vi "Paths.vi"(7 "error constant":errorcluster, 10 "file path (dialog if empty)":path) -> (0 "error IO":errorcluster, 1 "limits file path":path, 2 "File Names":string[](array[string]), 3 "All MCS Registers":cluster{"all rows":string[][]}[](array[cluster]), 4 "Calibration date file path":path, 5 "Email settings file path":path, 6 "Users Db":path, 8 "Limit of rate change path":path, 9 "Offsets file path":path)   [LabVIEW 2025]
uses:
  CTRLS/GLB_VAR.vi
  mcs/Tachometer_MAIN Folder/CTRLS/New/MCS Tag.ctl
  CTRLS/New/Monitiring MCS Tags.ctl
  CTRLS/New/Mcs All Tags Registers.ctl
  <vilib>/Utility/file.llb/Read Delimited Spreadsheet (string).vi
panel:
  out "Array 5":string[][](array[string])
  out "Array 4":string[][](array[string])
  out "Array 3":string[][](array[string])
  out "Array 2":i32[](array[numeric])
  out "Array":i32[](array[numeric])
  out "Register":string[](array[string])
  out "Name":string[](array[string])
  out "Application Directory":path
  out "Templates directory":path
  out "config file path":path
  out "Test Setups directory":path
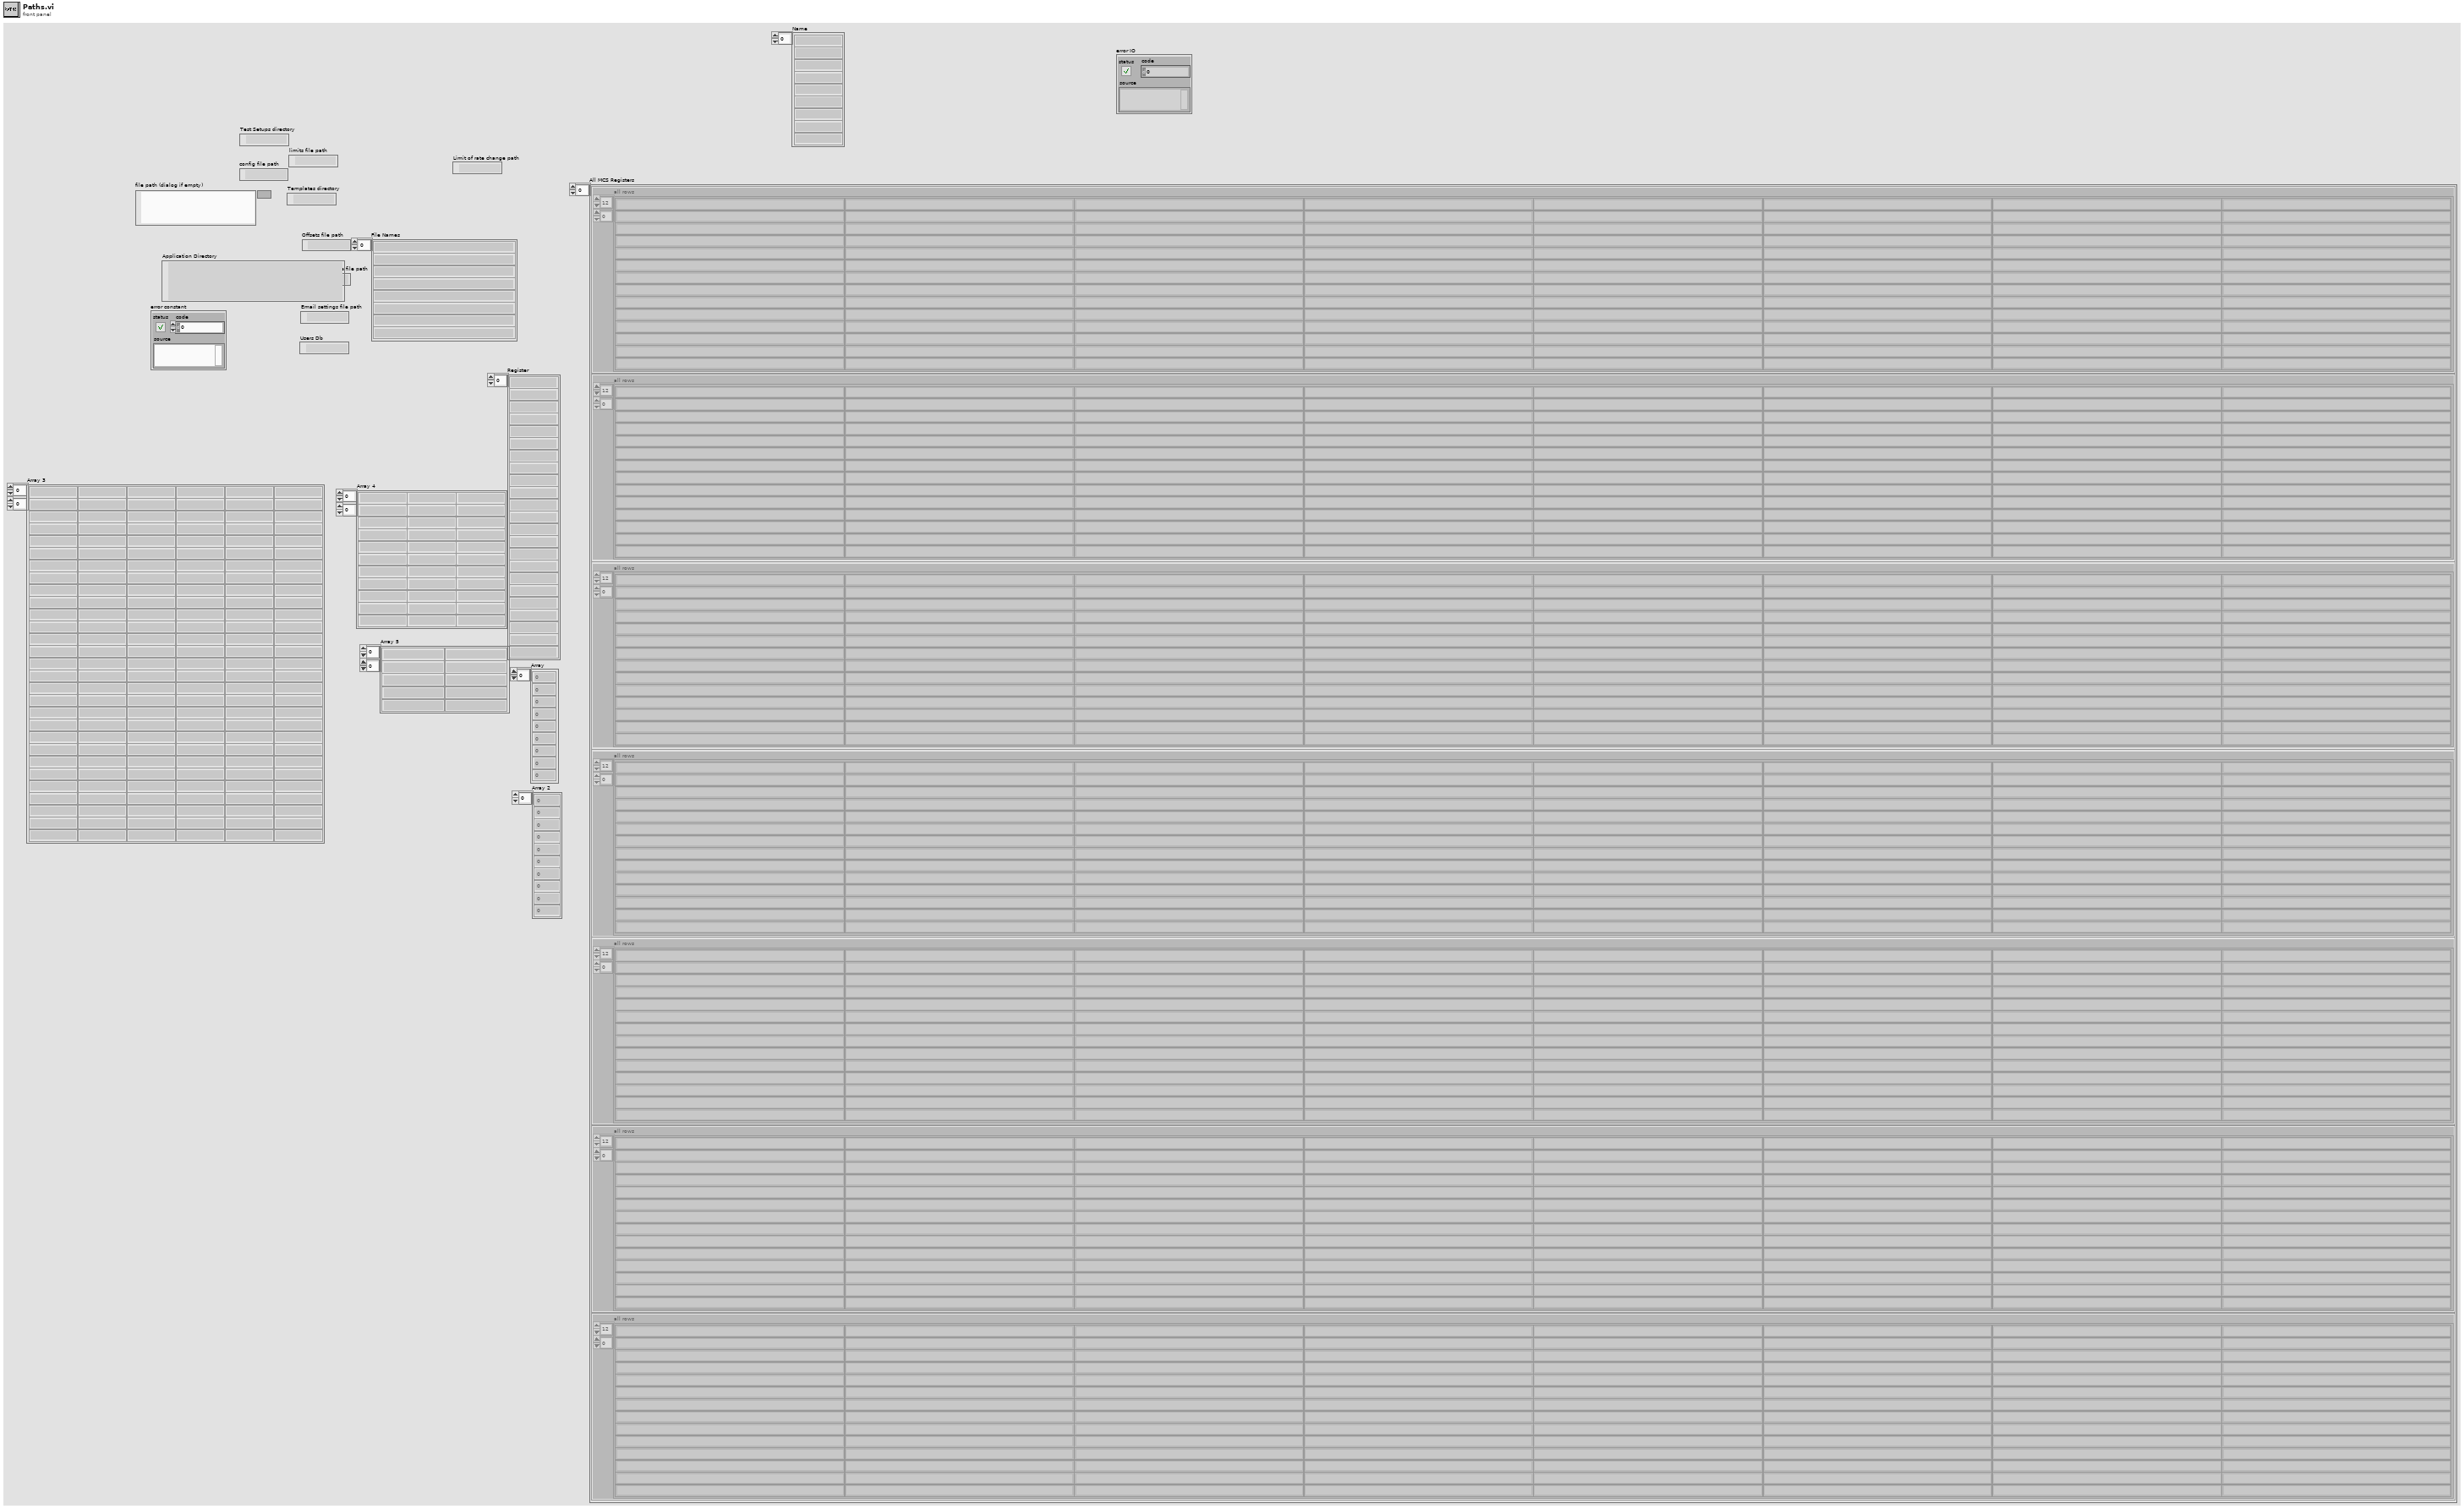
[diagram p1: front panel]
types:
  T1 = typedef "Mcs All Tags Registers.ctl" = cluster{"Suction addr":i32[][], "Discharge addr":i32[][], "Loging addr":i32[][], "Monitiring MCS Tags":T2, "Monitiring MCS Coils":cluster{"Tag Name":string, "Modbus Input Register":sgl, "Value":bool}[][]}
  T2 = typedef "Monitiring MCS Tags.ctl" = T3[][]
  T3 = typedef "MCS Tag.ctl" = cluster{"Tag Name":string, "Modbus Input Register":sgl, "Value":sgl}
  T4 = cluster{"Tag Name":string, "Modbus Input Register":sgl, "Value":bool}[][]
  T5 = enum16{"open", "replace", "create", "open or create", "replace or create", "replace or create with confirmation"}
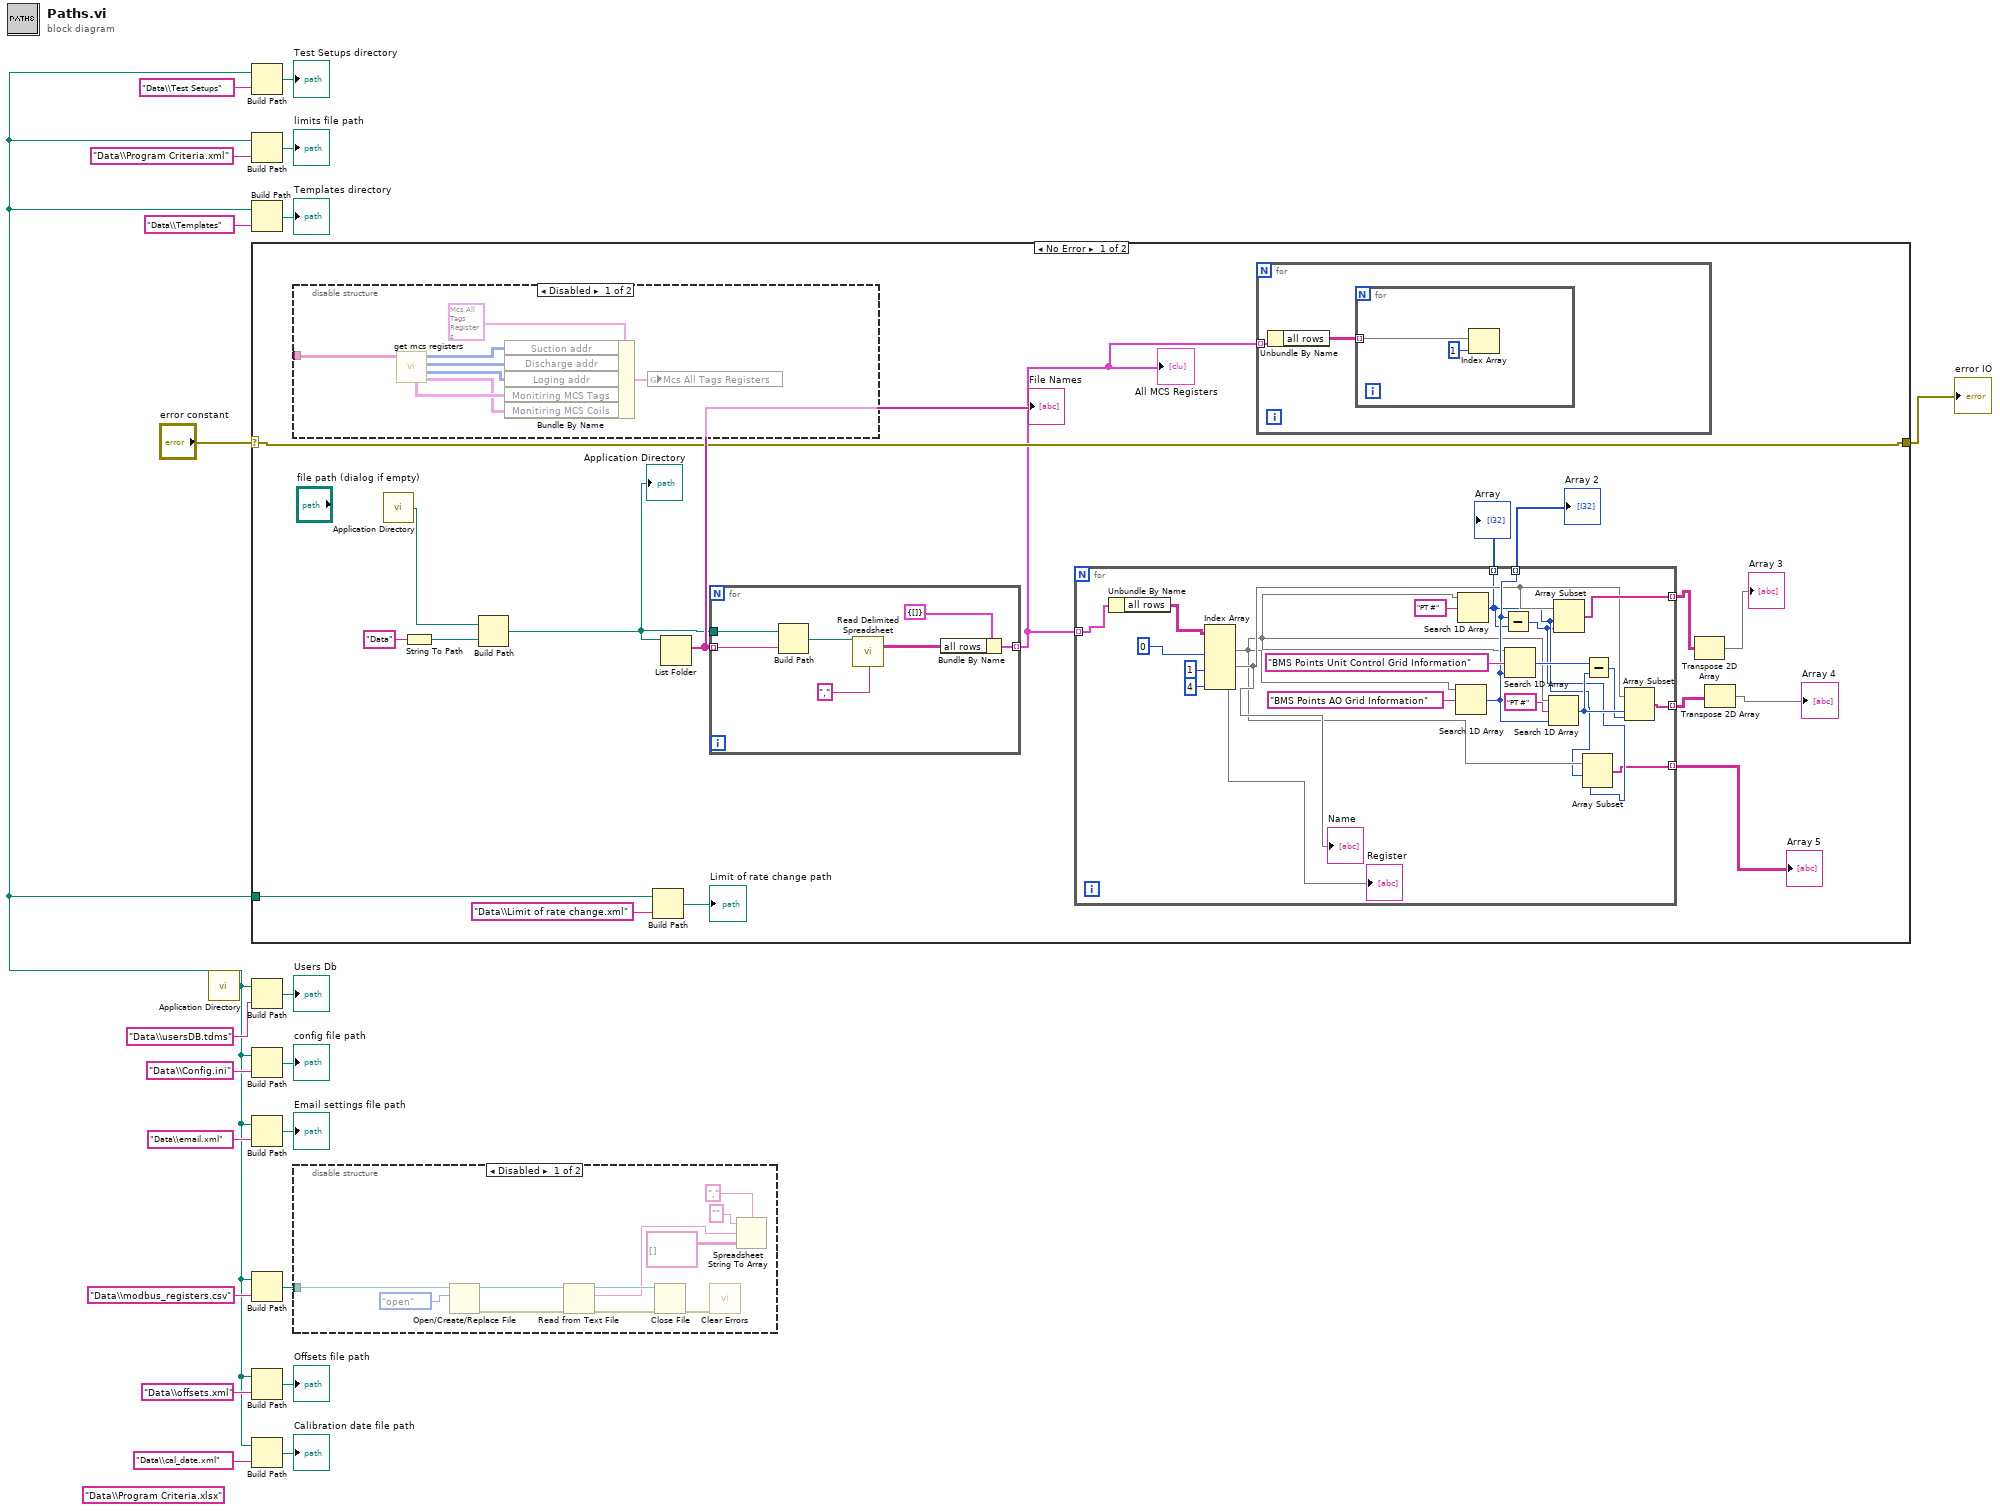
[diagram p0: block diagram]
diagram:
  (unwired) "Data\\Program Criteria.xlsx"
  n1 = call <vilib>:"Application Directory.vi"() -> ("Application Directory"=w4:path)
  n2 = Build Path(base path=w4, name or relative path="Data\\Test Setups") -> (appended path=→"Test Setups directory":path)
  n3 = Build Path(base path=w4, name or relative path="Data\\Program Criteria.xml") -> (appended path=→"limits file path":path)
  n4 = Build Path(base path=w4, name or relative path="Data\\Templates") -> (appended path=→"Templates directory":path)
  n5 = case shown="No Error" "error constant" {
    selector: "error constant" -> [w31 w79]
    tunnel: w4 -> [w36 _]
    tunnel: [w31 w79] -> w1
    frame No Error {
      n6 = disable-structure shown="Disabled" {
        disable-tunnel: _ -> [w75 _]
        frame Disabled {
          n7 = call "get mcs registers.vi"("MCS CSV"=w75) -> ("coils"=w73:T4, "Array 2"=w76:i32[][], "Array 3"=w77:i32[][], "Array 4"=w78:i32[][], "Array"=w74:T3[][])  [unwired: 6 in]
          n8 = Bundle By Name(cluster=T1 {"Suction addr"=[[30003, 30004, 30005, 30006], [30011, 30012, 30016, 30017], [30098, 30103, 30108, 30113], [30101, 30106, 30111, 30116]], "Discharge addr"=[[30007, 30008, 30009, 30010], [30018, 30019, 30020, 30021], [30099, 30104, 30109, 30114], [30100, 30105, 30110, 30115]], "Loging addr"=[[30093, 30094, 30095, 30096, 0, 0], [30097, 30102, 30107, 30112, 0, 0], [30087, 30088, 30089, 30090, 30091, 30092], [30036, 30037, 30038, 30039, 0, 0], [30001, 30002, 0, 0, 0, 0], [30044, 30045, 0, 0, 0, 0], [30117, 30118, 30119, 0, 0, 0], [30022, 30023, 30024, 30025, 30026, 30027]], "Monitiring MCS Tags"=[[{"Tag Name"="MP+OL1", "Modbus Input Register"=30028.0, "Value"=0.0}, {"Tag Name"="MP+OL2", "Modbus Input Register"=30029.0, "Value"=0.0}], [{"Tag Name"="MP+OL2", "Modbus Input Register"=30029.0, "Value"=0.0}, {"Tag Name"="MP+OL3", "Modbus Input Register"=30030.0, "Value"=0.0}], [{"Tag Name"="MP+OL3", "Modbus Input Register"=30030.0, "Value"=0.0}, {"Tag Name"="MP+OL4", "Modbus Input Register"=30031.0, "Value"=0.0}], [{"Tag Name"="MP+OL4", "Modbus Input Register"=30031.0, "Value"=0.0}, {"Tag Name"="OIL.LEVEL1", "Modbus Input Register"=30032.0, "Value"=0.0}], [{"Tag Name"="OIL.LEVEL1", "Modbus Input Register"=30032.0, "Value"=0.0}, {"Tag Name"="OIL.LEVEL2", "Modbus Input Register"=30033.0, "Value"=0.0}], [{"Tag Name"="OIL.LEVEL2", "Modbus Input Register"=30033.0, "Value"=0.0}, {"Tag Name"="OIL.LEVEL3", "Modbus Input Register"=30034.0, "Value"=0.0}], [{"Tag Name"="OIL.LEVEL3", "Modbus Input Register"=30034.0, "Value"=0.0}, {"Tag Name"="OIL.LEVEL4", "Modbus Input Register"=30035.0, "Value"=0.0}], [{"Tag Name"="OIL.LEVEL4", "Modbus Input Register"=30035.0, "Value"=0.0}, {"Tag Name"="PUMPDOWN1", "Modbus Input Register"=30040.0, "Value"=0.0}], [{"Tag Name"="PUMPDOWN1", "Modbus Input Register"=30040.0, "Value"=0.0}, {"Tag Name"="PUMPDOWN2", "Modbus Input Register"=30041.0, "Value"=0.0}], [{"Tag Name"="PUMPDOWN2", "Modbus Input Register"=30041.0, "Value"=0.0}, {"Tag Name"="PUMPDOWN3", "Modbus Input Register"=30042.0, "Value"=0.0}], [{"Tag Name"="PUMPDOWN3", "Modbus Input Register"=30042.0, "Value"=0.0}, {"Tag Name"="PUMPDOWN4", "Modbus Input Register"=30043.0, "Value"=0.0}], [{"Tag Name"="PUMPDOWN4", "Modbus Input Register"=30043.0, "Value"=0.0}, {"Tag Name"="COMP1", "Modbus Input Register"=30046.0, "Value"=0.0}], [{"Tag Name"="COMP1", "Modbus Input Register"=30046.0, "Value"=0.0}, {"Tag Name"="COMP2", "Modbus Input Register"=30050.0, "Value"=0.0}], [{"Tag Name"="COMP2", "Modbus Input Register"=30050.0, "Value"=0.0}, {"Tag Name"="COMP3", "Modbus Input Register"=30054.0, "Value"=0.0}], [{"Tag Name"="COMP3", "Modbus Input Register"=30054.0, "Value"=0.0}, {"Tag Name"="COMP4", "Modbus Input Register"=30058.0, "Value"=0.0}], [{"Tag Name"="COMP4", "Modbus Input Register"=30058.0, "Value"=0.0}, {"Tag Name"="LOADSOL1", "Modbus Input Register"=30047.0, "Value"=0.0}], [{"Tag Name"="LOADSOL1", "Modbus Input Register"=30047.0, "Value"=0.0}, {"Tag Name"="LOADSOL2", "Modbus Input Register"=30051.0, "Value"=0.0}], [{"Tag Name"="LOADSOL2", "Modbus Input Register"=30051.0, "Value"=0.0}, {"Tag Name"="LOADSOL3", "Modbus Input Register"=30055.0, "Value"=0.0}], [{"Tag Name"="LOADSOL3", "Modbus Input Register"=30055.0, "Value"=0.0}, {"Tag Name"="LOADSOL4", "Modbus Input Register"=30059.0, "Value"=0.0}], [{"Tag Name"="LOADSOL4", "Modbus Input Register"=30059.0, "Value"=0.0}, {"Tag Name"="UNLDSOL1", "Modbus Input Register"=30048.0, "Value"=0.0}], [{"Tag Name"="UNLDSOL1", "Modbus Input Register"=30048.0, "Value"=0.0}, {"Tag Name"="UNLDSOL2", "Modbus Input Register"=30052.0, "Value"=0.0}], [{"Tag Name"="UNLDSOL2", "Modbus Input Register"=30052.0, "Value"=0.0}, {"Tag Name"="UNLDSOL3", "Modbus Input Register"=30056.0, "Value"=0.0}], [{"Tag Name"="UNLDSOL3", "Modbus Input Register"=30056.0, "Value"=0.0}, {"Tag Name"="UNLDSOL4", "Modbus Input Register"=30060.0, "Value"=0.0}], [{"Tag Name"="UNLDSOL4", "Modbus Input Register"=30060.0, "Value"=0.0}, {"Tag Name"="ESV1", "Modbus Input Register"=30049.0, "Value"=0.0}], [{"Tag Name"="ESV1", "Modbus Input Register"=30049.0, "Value"=0.0}, {"Tag Name"="ESV2", "Modbus Input Register"=30053.0, "Value"=0.0}], [{"Tag Name"="ESV2", "Modbus Input Register"=30053.0, "Value"=0.0}, {"Tag Name"="ESV3", "Modbus Input Register"=30057.0, "Value"=0.0}]], "Monitiring MCS Coils"=[]} ("Mcs All Tags Registers"), "Suction addr"=w78, "Discharge addr"=w77, "Loging addr"=w76, "Monitiring MCS Tags"=w74, "Monitiring MCS Coils"=w73) -> (w71:T1)
          n9 = global write "GLB_VAR.vi" "Mcs All Tags Registers"(w71) -> ()
        }
        frame Enabled {
        }
      }
      n10 = call <vilib>:"Application Directory.vi"() -> ("Application Directory"=w23:path)
      n11 = String To Path(string="Data") -> (path=w34:path)
      n12 = Build Path(base path=w23, name or relative path=w34) -> (appended path=w32:path)
      "Application Directory" <- w32
      n13 = Build Path(base path=w36, name or relative path="Data\\Limit of rate change.xml") -> (appended path=→"Limit of rate change path":path)
      n14 = List Folder(path=w32) -> (filenames=w33:string[])  [unwired: 3 in, 3 out]
      "File Names" <- w33
      n15 = for {
        tunnel: w33 -> [w68] mode=indexing
        tunnel: w32 -> [w69]
        tunnel: [w64] -> w22 mode=indexing
        n16 = Build Path(base path=w69, name or relative path=w68) -> (appended path=w67:path)
        n17 = call-poly <vilib>:"Read Delimited Spreadsheet.vi"("file path (dialog if empty)"=w67, "delimiter (\\t)"="," ("delimiter (\\t)")) -> ("all rows"=w66:string[][])  [unwired: 8 in, 5 out]
        n18 = Bundle By Name(cluster=cluster{"all rows":string[][]} {"all rows"=[]}, "all rows"=w66) -> (w64:cluster{"all rows":string[][]})
      }
      "All MCS Registers" <- w22
      n19 = for {
        tunnel: w22 -> [w63] mode=indexing
        tunnel: [w45] -> w30 mode=indexing
        tunnel: [w52] -> w29 mode=indexing
        tunnel: [w55] -> w28 mode=indexing
        tunnel: [w47] -> w26 mode=indexing
        tunnel: [w43] -> w24 mode=indexing
        n20 = Unbundle By Name(w63) -> ("all rows"=w62:string[][])
        n21 = Index Array(array=w62, index (col) #1=0 ("disabled index (col)"), index (col) #2=1 ("index (col)"), index (col) #3=4 ("index (col)")) -> (element #1=w46:string[], element #2=w50:string[], element #3=→"Register":string[])  [unwired: 3 in]
        "Name" <- w50
        n22 = Search 1D Array(1D array=w46, element="BMS Points AO Grid Information") -> (index of element=w52:i32)  [unwired: 1 in]
        n23 = Search 1D Array(1D array=w46, element="PT #") -> (index of element=w45:i32)  [unwired: 1 in]
        n24 = Subtract(x=w52, y=w45) -> (x-y=w44:i32)
        n25 = Search 1D Array(1D array=w46, element="BMS Points Unit Control Grid Information", start index (0)=w52) -> (index of element=w51:i32)
        n26 = Search 1D Array(1D array=w46, element="PT #", start index (0)=w52) -> (index of element=w49:i32)
        n27 = Array Subset(array=w50, index=w45, length=w44) -> (w55:string[])
        n28 = Array Subset(array=w46, index=w45, length=w44) -> (w43:string[])
        n29 = Subtract(x=w51, y=w49) -> (x-y=w48:i32)
        n30 = Array Subset(array=w50, index=w49, length=w48) -> (w47:string[])
      }
      "Array" <- w30
      "Array 2" <- w29
      "Array 5" <- w24
      n31 = for {
        tunnel: w22 -> [w40] mode=indexing
        n32 = Unbundle By Name(w40) -> ("all rows"=w39:string[][])
        n33 = for {
          tunnel: w39 -> [w42] mode=indexing
          n34 = Index Array(array=w42, index=1) -> ()  [unwired: 1 out]
        }
      }
      n35 = Transpose 2D Array(2D array=w28) -> (transposed array=→"Array 3":string[][])
      n36 = Transpose 2D Array(2D array=w26) -> (transposed array=→"Array 4":string[][])
    }
    frame Error {
    }
  }
  "error IO" <- w1
  n37 = Build Path(base path=w4, name or relative path="Data\\usersDB.tdms") -> (appended path=→"Users Db":path)
  n38 = Build Path(base path=w4, name or relative path="Data\\Config.ini") -> (appended path=→"config file path":path)
  n39 = Build Path(base path=w4, name or relative path="Data\\email.xml") -> (appended path=→"Email settings file path":path)
  n40 = Build Path(base path=w4, name or relative path="Data\\modbus_registers.csv") -> (appended path=w3:path)
  n41 = Build Path(base path=w4, name or relative path="Data\\offsets.xml") -> (appended path=→"Offsets file path":path)
  n42 = Build Path(base path=w4, name or relative path="Data\\cal_date.xml") -> (appended path=→"Calibration date file path":path)
  n43 = disable-structure shown="Disabled" {
    disable-tunnel: w3 -> [w80 _]
    frame Disabled {
      n44 = Open/Create/Replace File(file path (use dialog)=w80, operation (0:open)=T5."open") -> (refnum out=w89:refnum<file>, error out=w88:errorcluster)  [unwired: 4 in, 1 out]
      n45 = Read from Text File(file (use dialog)=w89, error in=w88) -> (refnum out=w86:refnum<file>, text=w85:string, error out=w87:errorcluster)  [unwired: 2 in, 1 out]
      n46 = Close File(refnum=w86, error in=w87) -> (error out=w81:errorcluster)  [unwired: 1 out]
      n47 = call <vilib>:"Clear Errors.vi"("error in (no error)"=w81) -> ()  [unwired: 5 in, 2 out]
      n48 = Spreadsheet String To Array(delimiter (Tab)=",", format string="", spreadsheet string=w85, array type (2D Dbl)=string[][] []) -> ()  [unwired: 1 out]
    }
    frame Enabled {
    }
  }
